vi "Parse Response.vi"(8 "error in (no error)":errorcluster, 10 "<JSON> Response":string) -> (0 "error out":errorcluster, 1 "results":string, 4 "IDs":string)   [LabVIEW 2019, in "JSON-RPC.lvlib"]
doc: "Parse a Response object to extract an object's <b>result</b>, and <b>id</b>.\n\nThe <b>result</b> datatype is a JSON object and will need further processing to convert to LabVIEW data. It is formatted in the same way as a Request object's params.\n\nhttps://www.jsonrpc.org/specification"
uses:
  JSON-RPC.lvlib
  <vilib>/JDP Science/JSONtext/JSONtext.lvlib
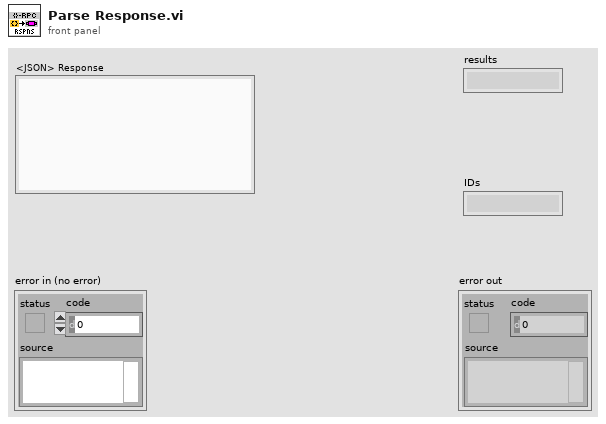
[diagram p1: front panel]
types:
  T1 = typedef "JSONtext.lvlib/JSON Value Type.ctl" = enum16{"Not a JSON Value", "JSON Object", "JSON Array", "String", "Number", "true", "false", "null"}
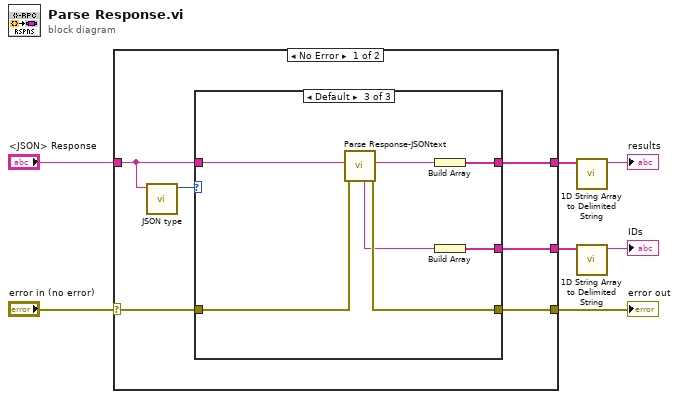
[diagram p0: block diagram]
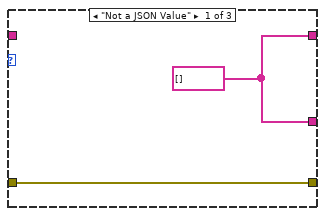
[diagram p2: hidden frame]
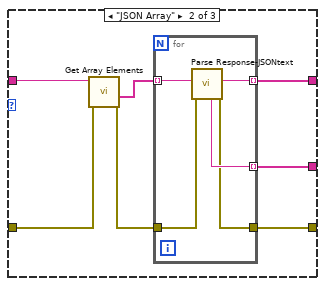
[diagram p3: hidden frame]
diagram:
  n1 = case shown="No Error" "error in (no error)" {
    selector: "error in (no error)" -> [w11 w35]
    tunnel: [w8 w35] -> w6
    tunnel: "<JSON> Response" -> [w12 _]
    tunnel: [w10 _] -> w2
    tunnel: [w9 _] -> w4
    frame No Error {
      n2 = call <vilib>:"JSON type.vi"("JSON"=w12) -> ("JSON Value Type"=w13:T1)  [unwired: 9 in, 1 out]
      n3 = case shown="Default" w13 {
        tunnel: w11 -> [w15 w19 w33]
        tunnel: [w15 w22 w32] -> w8
        tunnel: w12 -> [_ w20 w34]
        tunnel: [w14 w21 w30] -> w10
        tunnel: [w14 w18 w28] -> w9
        frame "Not a JSON Value" {
          w14 = string[] []
        }
        frame "JSON Array" {
          n4 = call <vilib>:"Get Array Elements.vi"("error in (no error)"=w19, "JSON"=w20) -> ("error out"=w16:errorcluster, "<JSON>"=w17:string[])  [unwired: 7 in, 1 out]
          n5 = for {
            tunnel: w17 -> [w27] mode=indexing
            tunnel: [w25] -> w21 mode=indexing
            tunnel: [w24] -> w18 mode=indexing
            tunnel: w16 -> [w26]
            tunnel: [w23] -> w22
            n6 = call "Parse Response-JSONtext.vi"("error in (no error)"=w26, "<JSON> Response"=w27) -> ("error out"=w23:errorcluster, "result"=w25:string, "id"=w24:string)  [unwired: 7 in]
          }
        }
        frame Default {
          n7 = call "Parse Response-JSONtext.vi"("error in (no error)"=w33, "<JSON> Response"=w34) -> ("error out"=w32:errorcluster, "result"=w31:string, "id"=w29:string)  [unwired: 7 in]
          n8 = Build Array(w31) -> (w30:string[])
          n9 = Build Array(w29) -> (w28:string[])
        }
      }
    }
    frame Error {
    }
  }
  "error out" <- w6
  n10 = call <vilib>:"1D String Array to Delimited String.vi"("string array"=w2) -> ("delimited string"=→"results":string)  [unwired: 10 in]
  n11 = call <vilib>:"1D String Array to Delimited String.vi"("string array"=w4) -> ("delimited string"=→"IDs":string)  [unwired: 10 in]
